vi "SysDef.Compile.vi"(8 "error in (no error)":errorcluster, 11 "Device Reference in":T1 format="%.0x") -> (0 "error out":errorcluster, 1 "Refs":T2(array[cluster]) {"VS Refs" format="%.0x"}, 2 "VS References":T3={"Name"="", "CAN"={"Interface"="", "Baud Rate"=0, "Diagnostic Protocol"=enum."GMLAN", "Transport Protocol"=enum."ISO TP - Normal Mode", "Transmit ID"=0, "Receive ID"=2, "Transmit Extension"=1, "Receive Extension"=255, "Receive UUDT ID"=0, "Enable Stream"=TRUE, "VW TP Channel ID"=1, "Fill Frame"=FALSE, "Fill Byte"=0, "Termination"=FALSE, "LIN Cluster"="", "NAD"=8, "IO Mode"=0, "Max DLC"=0, "FD Baud Rate"=2, "Timeout"=1, "FD ISO Mode"=0, "DoIP Address"="", "DoIP Source Address"=3584, "DoIP Dynamic Port"=TRUE, "DoIP Version"=2}, "986x"={"Enable"=FALSE, "RIO Device"="", "Bitfile"=path ""}, "Reads"=[], "Frames Lookup"=variant(enum16{"GMLAN", "KWP-2000", "UDS"} enum."GMLAN"), "Writes"=[], "DPIDs"=[], "DPID Lookup"=variant(u32 0), "DTC"={"Descriptor"={"DTC Byte Length"=1, "Status Byte Length"=1, "Add Data Byte Length"=1, "Byte Order"=enum."Motorola"}, "Value.Code"=[], "Value.String"=[], "Value.J2012String"=[], "Status.Code"=[], "Status.String"=[]}, "Created DTCs"=0, "Polls"=[], "Service Channels Status Lookup"=variant, "Trigger Lookup"=variant, "Security"={"Type"=enum."None", "Source DLL Path"=path "", "Target DLL Path"=path "", "Security Level"=1, "Static Master Key"="", "Max Key Length"=1, "Host IP Address"="", "ECU  Variant"=0, "Optional Parameter"=0}, "Initial Comm State"=FALSE} {"Writes"."Signals"."Byte Order" items=["Little Endian", "Big Endian"]; "Writes"."Signals"."Data Type" items=["Signed", "Unsigned", "IEEE Float"]; "CAN"."DoIP Version" items=["2010"=1, "2012"=2]; "CAN"."DoIP Source Address" format="%.0x"; "CAN"."FD ISO Mode" items=["ISO", "Non ISO", "ISO Legacy"]; "CAN"."IO Mode" items=["CAN 2.0", "CAN FD", "CAN FD+BRS"]; "CAN"."Fill Byte" format="%.0x"; "CAN"."VW TP Channel ID" format="%.0x"; "CAN"."Receive UUDT ID" format="%.0x"; "CAN"."Receive Extension" format="%.0x"; "CAN"."Transmit Extension" format="%.0x"; "CAN"."Receive ID" format="%.0x"; "CAN"."Transmit ID" format="%.0x"; "Reads"."Signals"."Byte Order" items=["Little Endian", "Big Endian"]; "Reads"."Signals"."Data Type" items=["Signed", "Unsigned", "IEEE Float"]}, 3 "Device Reference out":T1 format="%.0x")   [LabVIEW 2024, in "Diagnostics Addon System Explorer.lvlib"]
uses:
  Diagnostics Addon System Explorer.lvlib
  <vilib>/NI VeriStand/Custom Device API/Custom Device Item Ref.ctl
  Addon Shared/Types/SysDef.Compile.ctl
  Addon Shared/Types/CAN.ctl
  Addon Shared/Types/CAN.Interface.ctl
  Addon Shared/Types/Protocol.ctl
  Addon Shared/Types/Transport.ctl
  Addon Shared/Types/986x.ctl
  Addon Shared/Types/Frame.Compile.ctl
  Addon Shared/Types/Type.ctl
  Addon Shared/Types/Signal.ctl
  Addon Shared/Types/DPID.ctl
  Addon Shared/Types/DPID.Rate.ctl
  Addon Shared/Types/DTC.Settings.ctl
  Addon Shared/Types/DTC.Descriptor.ctl
  Addon Shared/Types/Poll.Compiled.ctl
  Addon Shared/Types/Security.ctl
  Addon Shared/Types/Security.Type.ctl
  Types/FG.Action.ctl
  ID.FG.vi
  Signals.Get.vi
  Type.FG.vi
  ServiceChannels.GetRefs.vi
  SettingChannels.GetRefs.vi
  Addon Shared/SubVIs/Frame.Get.Size.vi
  Addon Shared/SubVIs/LookupID.Create.vi
  DPID.FG.vi
  Security.FG.vi
  Signal.FG.vi
  Frame.GetSignalRefs.vi
  FileDependency.Create.vi
  Addon Shared/SubVIs/Constants.vi
  <vilib>/NI VeriStand/Custom Device Tools/Custom Device Utility Library/NI VeriStand - Search for Item by GUID.vi
  <vilib>/NI VeriStand/Custom Device Tools/Custom Device Utility Library/NI VeriStand - Search for Item by Name.vi
  <vilib>/NI VeriStand/Custom Device API/NI VeriStand - Get Item Children.vi
  <vilib>/NI/NI VeriStand Advanced SysDef API/SysDef API/SysDef.Property.Set.vi
  <vilib>/NI/NI VeriStand Advanced SysDef API/_SubVIs/SysDef.Property.Set.U32.vi
  <vilib>/NI VeriStand/Custom Device API/NI VeriStand - Get Item Property.vi
  <vilib>/NI VeriStand/Custom Device API/Get Item Property (U32).vi
  <vilib>/NI/NI VeriStand Advanced SysDef API/_SubVIs/SysDef.Property.Set.DBL.vi
  <vilib>/NI/NI VeriStand Advanced SysDef API/_SubVIs/SysDef.Property.Set.String.vi
  <vilib>/NI VeriStand/Custom Device API/Get Item Property (Double).vi
  <vilib>/NI VeriStand/Custom Device API/Get Item Property (String).vi
  <vilib>/NI VeriStand/Custom Device API/NI VeriStand - Get Custom Device Channel Data.vi
  <vilib>/NI VeriStand/Custom Device Tools/Custom Device Utility Library/NI VeriStand - Search for All Items by GUID.vi
  <vilib>/NI VeriStand/Custom Device API/Get Item Property (Variant).vi
  <vilib>/NI VeriStand/Custom Device API/Get Item Property (Boolean).vi
  <vilib>/NI VeriStand/Custom Device API/Get Item Property (U16).vi
  <vilib>/NI/NI VeriStand Advanced SysDef API/_SubVIs/SysDef.Property.Set.Variant.vi
  <vilib>/NI/NI VeriStand Advanced SysDef API/_SubVIs/SysDef.Property.Set.Boolean.vi
  <vilib>/NI/NI VeriStand Advanced SysDef API/_SubVIs/SysDef.Property.Set.U16.vi
  Service.EnumToGUID.vi
  <vilib>/NI VeriStand/Custom Device API/Get Item Property (Path).vi
  FileDependency.Get.Target Path.vi
  <vilib>/NI VeriStand/Custom Device API/Get Item Property (I32).vi
  <vilib>/NI/NI VeriStand Advanced SysDef API/SysDef API/SysDef.Property.Remove.vi
  <vilib>/NI/NI VeriStand Advanced SysDef API/_SubVIs/SysDef.Property.Set.Path.vi
  <vilib>/Utility/MD5Checksum.llb/MD5Checksum File.vi
  <vilib>/NI/NI VeriStand Advanced SysDef API/_SubVIs/SysDef.Property.Set.DependentFile.vi
  <vilib>/NI/NI VeriStand Advanced SysDef API/_SubVIs/SysDef.Property.Set.I32.vi
  <vilib>/NI/NI VeriStand Advanced SysDef API/_SubVIs/SysDef.Property.Set.U32.Array.vi
  <vilib>/NI VeriStand/Custom Device API/Get Item Property (U32 Array).vi
  Poll.FG.vi
  <vilib>/NI/NI VeriStand Advanced SysDef API/_SubVIs/SysDef.Property.Set.DBL.Array.vi
  <vilib>/NI/NI VeriStand Advanced SysDef API/_SubVIs/SysDef.Property.Set.String.Array.vi
  <vilib>/NI VeriStand/Custom Device API/Get Item Property (Double Array).vi
  <vilib>/NI VeriStand/Custom Device API/Get Item Property (String Array).vi
  <vilib>/NI VeriStand/Custom Device Tools/Custom Device Utility Library/Custom Device Utility Library.lvlib
  Addon Shared/Diagnostics Addon Shared.lvlib
  <vilib>/NI VeriStand/Custom Device API/Custom Device API.lvlib
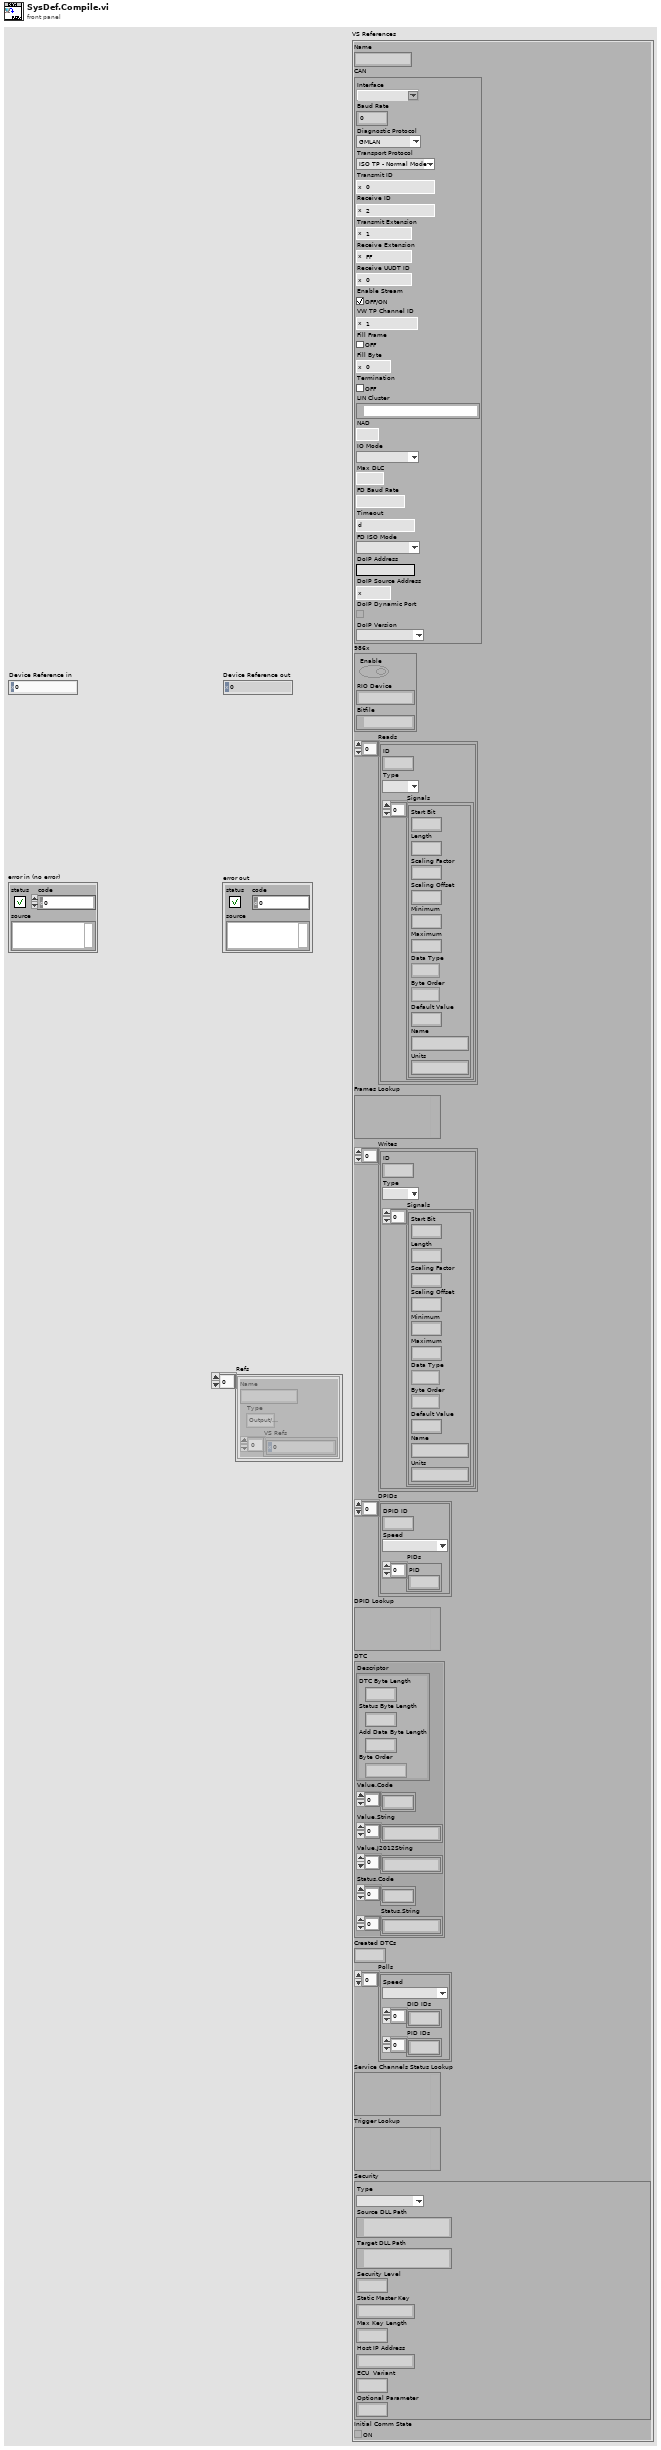
[diagram p1: front panel]
types:
  T1 = typedef "Custom Device API.lvlib/Custom Device Item Ref.ctl" = u64
  T2 = cluster{"Name":string, "Type":enum16{"Output/Write", "Input/Read", "Input/ReadWrite"}, "VS Refs":T1[]}[]
  T3 = typedef "Diagnostics Addon Shared.lvlib/SysDef.Compile.ctl" = cluster{"Name":string, "CAN":T4, "986x":T8, "Reads":T9[], "Frames Lookup":variant, "Writes":T9[], "DPIDs":T12[], "DPID Lookup":variant, "DTC":T14, "Created DTCs":u32, "Polls":T16[], "Service Channels Status Lookup":variant, "Trigger Lookup":variant, "Security":T17, "Initial Comm State":bool}
  T4 = typedef "Diagnostics Addon Shared.lvlib/CAN.ctl" = cluster{"Interface":T5, "Baud Rate":u64, "Diagnostic Protocol":T6, "Transport Protocol":T7, "Transmit ID":u32, "Receive ID":u32, "Transmit Extension":u8, "Receive Extension":u8, "Receive UUDT ID":u32, "Enable Stream":bool, "VW TP Channel ID":u32, "Fill Frame":bool, "Fill Byte":u8, "Termination":bool, "LIN Cluster":refnum<k21>, "NAD":u8, "IO Mode":u32, "Max DLC":u16, "FD Baud Rate":u64, "Timeout":u32, "FD ISO Mode":u32, "DoIP Address":string, "DoIP Source Address":u16, "DoIP Dynamic Port":bool, "DoIP Version":u16}
  T5 = typedef "Diagnostics Addon Shared.lvlib/CAN.Interface.ctl" = string
  T6 = typedef "Diagnostics Addon Shared.lvlib/Protocol.ctl" = enum16{"GMLAN", "KWP-2000", "UDS", "User-Defined"}
  T7 = typedef "Diagnostics Addon Shared.lvlib/Transport.ctl" = enum16{"ISO TP - Normal Mode", "ISO TP - Mixed Mode", "VW TP 2.0", "Diagnostics on IP", "ISO TP LIN"}
  T8 = typedef "Diagnostics Addon Shared.lvlib/986x.ctl" = cluster{"Enable":bool, "RIO Device":string, "Bitfile":path}
  T9 = typedef "Diagnostics Addon Shared.lvlib/Frame.Compile.ctl" = cluster{"ID":u32, "Type":T10, "Signals":T11[]}
  T10 = typedef "Diagnostics Addon Shared.lvlib/Type.ctl" = enum16{"DID", "CDID", "PID", "CPID", "Read Memory", "Write Memory", "IO Control", "Routine Start", "Routine Request", "Routine Stop", "User Defined", "DTC Control", "Clear DTCs", "Read DTCs", "Start DTCs", "DTC Change Count", "Tester Present", "Unlock ECU", "Reset ECU", "Diag Session Control", "Communication Control", "DPID Control", "Poll Control", "Diag Comm Port Control"}
  T11 = typedef "Diagnostics Addon Shared.lvlib/Signal.ctl" = cluster{"Start Bit":u32, "Length":u32, "Scaling Factor":dbl, "Scaling Offset":dbl, "Minimum":dbl, "Maximum":dbl, "Data Type":u32, "Byte Order":u32, "Default Value":dbl, "Name":string, "Units":string}
  T12 = typedef "Diagnostics Addon Shared.lvlib/DPID.ctl" = cluster{"DPID ID":u8, "Speed":T13, "PIDs":u16[]}
  T13 = typedef "Diagnostics Addon Shared.lvlib/DPID.Rate.ctl" = enum16{"Slow", "Medium", "Fast"}
  T14 = typedef "Diagnostics Addon Shared.lvlib/DTC.Settings.ctl" = cluster{"Descriptor":T15, "Value.Code":dbl[], "Value.String":string[], "Value.J2012String":string[], "Status.Code":dbl[], "Status.String":string[]}
  T15 = typedef "Diagnostics Addon Shared.lvlib/DTC.Descriptor.ctl" = cluster{"DTC Byte Length":i32, "Status Byte Length":i32, "Add Data Byte Length":i32, "Byte Order":enum16{"Motorola", "Intel"}}
  T16 = typedef "Diagnostics Addon Shared.lvlib/Poll.Compiled.ctl" = cluster{"Speed":T13, "DID IDs":u32[], "PID IDs":u32[]}
  T17 = typedef "Diagnostics Addon Shared.lvlib/Security.ctl" = cluster{"Type":T18, "Source DLL Path":path, "Target DLL Path":path, "Security Level":u32, "Static Master Key":string, "Max Key Length":u32, "Host IP Address":string, "ECU  Variant":i8, "Optional Parameter":i8}
  T18 = typedef "Diagnostics Addon Shared.lvlib/Security.Type.ctl" = enum16{"None", "SeedKey DLL", "MasterKey (Channel)", "MasterKey (Static)", "SeedKey DLL (Windows)"}
  T19 = enum16{"Output/Write", "Input/Read", "Input/ReadWrite"}
  T20 = cluster{"Name":string, "Type":enum16{"Output/Write", "Input/Read", "Input/ReadWrite"}, "VS Refs":T1[]}
  T21 = typedef "Diagnostics Addon System Explorer.lvlib/FG.Action.ctl" = enum16{"Get", "Set"}
  T22 = typedef "Diagnostics Addon System Explorer.lvlib/Service.Export.ctl" = cluster{"Signal.Cmd.Refs":T23[], "Signal.Cmd.Info":T9[], "Signal.Resp.Refs":T23[], "Signal.Resp.Info":T9[], "Trigger.Refs":T23[], "Status.Refs":T23[], "Settings.Refs":T23[]}
  T23 = typedef "Diagnostics Addon System Explorer.lvlib/Frame.Ref.ctl" = cluster{"Type":T10, "ID":u32, "Signal Refs":T1[]}
  T24 = typedef "Custom Device API.lvlib/Custom Device Item Info.ctl" = cluster{"Name":string, "Is Channel":bool, "GUID":string, "Is Waveform":bool}
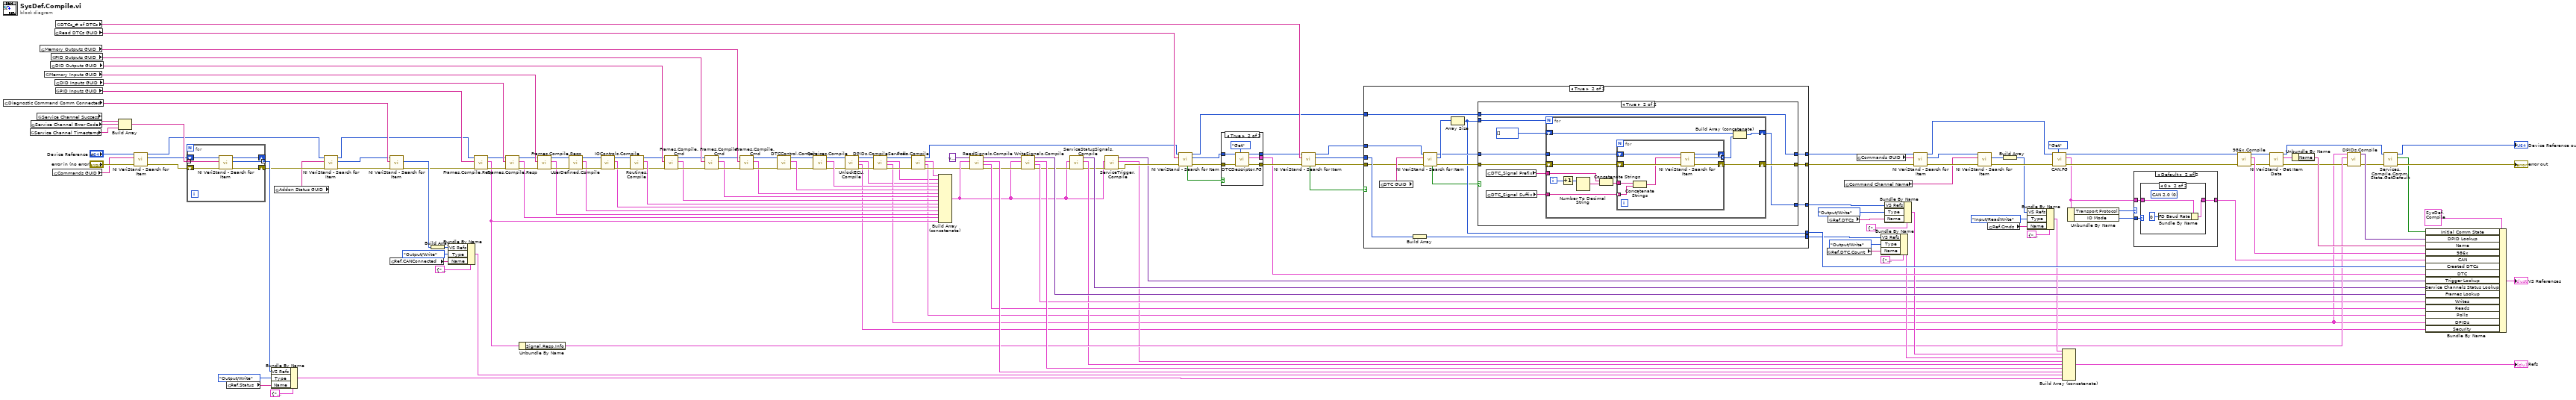
[diagram p0: block diagram]
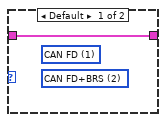
[diagram p3: hidden frame]
diagram:
  n1 = global read "Constants.vi" "Diagnostic Command Comm Connected"() -> (w76:string)
  n2 = global read "Constants.vi" "Service Channel Timestamp"() -> (w19:string)
  n3 = global read "Constants.vi" "Service Channel Error Code"() -> (w20:string)
  n4 = global read "Constants.vi" "Service Channel Success"() -> (w18:string)
  n5 = global read "Constants.vi" "Memory Outputs GUID"() -> (w133:string)
  n6 = global read "Constants.vi" "Memory Inputs GUID"() -> (w132:string)
  n7 = global read "Constants.vi" "DID Outputs GUID"() -> (w114:string)
  n8 = global read "Constants.vi" "PID Outputs GUID"() -> (w152:string)
  n9 = global read "Constants.vi" "Commands GUID"() -> (w67:string)
  n10 = global read "Constants.vi" "Read DTCs GUID"() -> (w156:string)
  n11 = global read "Constants.vi" "DID Inputs GUID"() -> (w153:string)
  n12 = global read "Constants.vi" "PID Inputs GUID"() -> (w151:string)
  n13 = global read "Constants.vi" "DTCs_# of DTCs"() -> (w155:string)
  n14 = Build Array(w18, w20, w19) -> (w118:string[])
  n15 = call-poly <vilib>:"NI VeriStand - Search for Item.vi"("error in"="error in (no error)", "Item GUID"=w67, "Section Ref in"="Device Reference in") -> ("error out"=w11:errorcluster, "Item Ref"=w10:T1, "Section Ref out"=w15:T1)  [unwired: 5 in, 1 out]
  n16 = for {
    tunnel: w118 -> [w160] mode=indexing
    tunnel: [w159] -> w96 mode=indexing
    shift-right: [w158] -> w17
    shift-left: w11 -> [w162]
    shift-right: [w157] -> _
    shift-left: w10 -> [w161]
    n17 = call-poly <vilib>:"NI VeriStand - Search for Item.vi"("error in"=w162, "Item Name"=w160, "Section Ref in"=w161) -> ("error out"=w158:errorcluster, "Item Ref"=w159:T1, "Section Ref out"=w157:T1)  [unwired: 5 in, 1 out]
  }
  n18 = global read "Constants.vi" "Ref.Status"() -> (w104:string)
  n19 = Bundle By Name(cluster=T20 {"Name"="", "Type"=enum."Output/Write", "VS Refs"=[]} ("Group"), "VS Refs"=w96, "Type"=T19."Output/Write", "Name"=w104) -> (w92:T20)
  n20 = global read "Constants.vi" "Addon Status GUID"() -> (w12:string)
  n21 = call-poly <vilib>:"NI VeriStand - Search for Item.vi"("error in"=w17, "Item GUID"=w12, "Section Ref in"=w15) -> ("error out"=w16:errorcluster, "Item Ref"=w13:T1, "Section Ref out"=w14:T1)  [unwired: 5 in, 1 out]
  n22 = call-poly <vilib>:"NI VeriStand - Search for Item.vi"("error in"=w16, "Item Name"=w76, "Section Ref in"=w13) -> ("error out"=w71:errorcluster, "Item Ref"=w73:T1)  [unwired: 5 in, 2 out]
  n23 = global read "Constants.vi" "Ref.CANConnected"() -> (w75:string)
  n24 = Build Array(w73) -> (w72:T1[])
  n25 = Bundle By Name(cluster=T20 {"Name"="", "Type"=enum."Output/Write", "VS Refs"=[]} ("Group"), "VS Refs"=w72, "Type"=T19."Output/Write", "Name"=w75) -> (w66:T20)
  n26 = call "Frames.Compile.Resp.vi"("error in (no error)"=w71, "GUID"=w151, "Section Ref in"=w14) -> ("error out"=w126:errorcluster, "Settings"=w61:T22, "Section Ref out"=w131:T1)  [unwired: 6 in]
  n27 = call "Frames.Compile.Resp.vi"("error in (no error)"=w126, "GUID"=w153, "Section Ref in"=w131) -> ("error out"=w127:errorcluster, "Settings"=w62:T22, "Section Ref out"=w130:T1)  [unwired: 6 in]
  n28 = Unbundle By Name(w61) -> ("Signal.Resp.Info"=w65:T9[])
  n29 = call "Frames.Compile.Resp.vi"("error in (no error)"=w127, "GUID"=w132, "Section Ref in"=w130) -> ("error out"=w112:errorcluster, "Settings"=w63:T22, "Section Ref out"=w113:T1)  [unwired: 6 in]
  n30 = call "UserDefined.Compile.vi"("error in (no error)"=w112, "Section Ref in"=w113) -> ("error out"=w111:errorcluster, "Settings"=w59:T22, "Section Ref out"=w110:T1)  [unwired: 7 in]
  n31 = call "IOControls.Compile.vi"("error in (no error)"=w111, "Section Ref in"=w110) -> ("error out"=w128:errorcluster, "Settings"=w58:T22, "Section Ref out"=w129:T1)  [unwired: 7 in]
  n32 = call "Routines.Compile.vi"("error in (no error)"=w128, "Section Ref in"=w129) -> ("error out"=w52:errorcluster, "Settings"=w57:T22, "Section Ref out"=w51:T1)  [unwired: 7 in]
  n33 = call "Frames.Compile.Cmd.vi"("error in (no error)"=w52, "GUID"=w114, "Section Ref in"=w51) -> ("error out"=w115:errorcluster, "Settings"=w53:T22, "Section Ref out"=w116:T1)  [unwired: 6 in]
  n34 = call "Frames.Compile.Cmd.vi"("error in (no error)"=w115, "GUID"=w152, "Section Ref in"=w116) -> ("error out"=w120:errorcluster, "Settings"=w54:T22, "Section Ref out"=w123:T1)  [unwired: 6 in]
  n35 = call "Frames.Compile.Cmd.vi"("error in (no error)"=w120, "GUID"=w133, "Section Ref in"=w123) -> ("error out"=w121:errorcluster, "Settings"=w55:T22, "Section Ref out"=w122:T1)  [unwired: 6 in]
  n36 = call "DTCControl.Compile.vi"("error in (no error)"=w121, "Section Ref in"=w122) -> ("error out"=w41:errorcluster, "Settings"=w56:T22, "Section Ref out"=w40:T1)  [unwired: 7 in]
  n37 = call "Services.Compile.vi"("error in (no error)"=w41, "Section Ref in"=w40) -> ("error out"=w25:errorcluster, "Settings"=w39:T22[], "Section Ref out"=w26:T1)  [unwired: 7 in]
  n38 = call "UnlockECU.Compile.vi"("error in (no error)"=w25, "Section Ref in"=w26) -> ("error out"=w24:errorcluster, "Security"=w21:T17, "Settings"=w22:T22[], "Section Ref out"=w23:T1)  [unwired: 6 in]
  n39 = call "DPIDs.CompileServices.vi"("error in (no error)"=w24, "Section Ref in"=w23) -> ("error out"=w32:errorcluster, "DPIDs Settings"=w28:T12[], "Settings"=w30:T22, "Section Ref out"=w31:T1)  [unwired: 6 in]
  n40 = call "Polls.Compile.vi"("error in (no error)"=w32, "Section Ref in"=w31) -> ("error out"=w36:errorcluster, "Poll Settings"=w33:T16[], "Service Channels"=w34:T22[], "Section Ref out"=w35:T1)  [unwired: 6 in]
  n41 = Build Array (concatenate)(w34, w30, w22, w39, w56, w55, w54, w53, w57, w58, w59, w63, w62, w61) -> (w44:T22[])
  n42 = call "ReadSignals.Compile.vi"("error in (no error)"=w36, "Settings"=w44, "Lookups in"=variant) -> ("error out"=w50:errorcluster, "Signal Info"=w64:T9[], "Refs"=w93:T20, "Lookups"=w101:variant)  [unwired: 5 in]
  n43 = call "WriteSignals.Compile.vi"("error in (no error)"=w50, "Settings"=w44, "Lookup In"=w101) -> ("error out"=w49:errorcluster, "Signal Info"=w60:T9[], "Refs"=w94:T20, "Lookup"=w100:variant)  [unwired: 5 in]
  n44 = call "ServiceStatusSignals.Compile.vi"("error in (no error)"=w49, "Settings"=w44) -> ("error out"=w46:errorcluster, "Refs"=w48:T20, "Status Lookup"=w47:variant)  [unwired: 7 in]
  n45 = call "ServiceTrigger.Compile.vi"("error in (no error)"=w46, "Settings"=w44) -> ("error out"=w45:errorcluster, "Refs"=w43:T2, "Trigger Lookup"=w42:variant)  [unwired: 7 in]
  n46 = call-poly <vilib>:"NI VeriStand - Search for Item.vi"("error in"=w45, "Item GUID"=w156, "Section Ref in"=w35) -> ("error out"=w147:errorcluster, "Item Ref"=w145:T1, "Section Ref out"=w117:T1, "Found"=w107:bool)  [unwired: 5 in]
  n47 = case shown="True" w107 {
    tunnel: w147 -> [w164 w169]
    tunnel: [w164 w168] -> w146
    tunnel: w145 -> [w163 w167]
    tunnel: [w163 w166] -> w144
    tunnel: [_ w165] -> w143
    frame False {
    }
    frame True {
      n48 = call "DTCDescriptor.FG.vi"("Action"=FG.Action."Get", "error in (no error)"=w169, "Device Item Ref in"=w167) -> ("error out"=w168:errorcluster, "DTC descriptor"=w165:T14, "Device Item Ref out"=w166:T1)  [unwired: 6 in]
    }
  }
  n49 = call-poly <vilib>:"NI VeriStand - Search for Item.vi"("error in"=w146, "Item Name"=w155, "Section Ref in"=w144) -> ("error out"=w149:errorcluster, "Item Ref"=w150:T1, "Section Ref out"=w109:T1, "Found"=w106:bool)  [unwired: 5 in]
  n50 = case shown="True" w106 {
    tunnel: w150 -> [_ w176]
    tunnel: w149 -> [w171 w175]
    tunnel: [_ w186] -> w86
    tunnel: [w171 w185] -> w125
    tunnel: [w172 w184] -> w124
    tunnel: w117 -> [w172 w174]
    tunnel: w109 -> [_ w181]
    tunnel: [_ w178] -> w108
    tunnel: [_ w173] -> w82
    frame False {
    }
    frame True {
      n51 = global read "Constants.vi" "DTC GUID"() -> (w179:string)
      n52 = Build Array(w176) -> (w173:T1[])
      n53 = call-poly <vilib>:"NI VeriStand - Search for Item.vi"("error in"=w175, "Item GUID"=w179, "Section Ref in"=w181) -> ("error out"=w183:errorcluster, "Item Refs"=w182:T1[], "Section Ref out"=w180:T1, "Found"=w177:bool)  [unwired: 5 in]
      n54 = Array Size(array=w182) -> (size(s)=w178:i32)
      n55 = case shown="True" w177 {
        tunnel: [_ w189] -> w186
        tunnel: [w187 w191] -> w185
        tunnel: [w188 w190] -> w184
        tunnel: w174 -> [w188 w190]
        tunnel: w183 -> [w187 w194]
        tunnel: w180 -> [_ w193]
        tunnel: w178 -> [_ w192]
        frame False {
        }
        frame True {
          n56 = global read "Constants.vi" "DTC_Signal Prefix"() -> (w197:string)
          n57 = global read "Constants.vi" "DTC_Signal Suffix"() -> (w196:string[])
          n58 = for {
            N: w192 -> [_]
            tunnel: w193 -> [w209]
            shift-right: [w207] -> w191
            shift-left: w194 -> [w208]
            tunnel: w196 -> [w202]
            tunnel: w197 -> [w201]
            shift-right: [w198] -> w189
            shift-left: T1[] [] -> [w200]
            i -> [w204]
            n59 = Increment(x=w204) -> (x+1=w206:i32)
            n60 = Number To Decimal String(number=w206) -> (decimal integer string=w205:string)  [unwired: 1 in]
            n61 = Concatenate Strings(w201, w205) -> (w203:string)
            n62 = for {
              shift-right: [w216] -> _
              shift-left: w209 -> [w217]
              shift-right: [w214] -> w207
              shift-left: w208 -> [w215]
              tunnel: w202 -> [w213] mode=indexing
              tunnel: w203 -> [w212]
              tunnel: [w210] -> w199 mode=indexing
              n63 = Concatenate Strings(w212, w213) -> (w211:string)
              n64 = call-poly <vilib>:"NI VeriStand - Search for Item.vi"("error in"=w215, "Item Name"=w211, "Section Ref in"=w217) -> ("error out"=w214:errorcluster, "Item Ref"=w210:T1, "Section Ref out"=w216:T1)  [unwired: 5 in, 1 out]
            }
            n65 = Build Array (concatenate)(w200, w199) -> (w198:T1[])
          }
        }
      }
    }
  }
  n66 = global read "Constants.vi" "Ref.DTC.Count"() -> (w84:string)
  n67 = global read "Constants.vi" "Ref.DTCs"() -> (w89:string)
  n68 = global read "Constants.vi" "Command Channel Name"() -> (w78:string)
  n69 = global read "Constants.vi" "Commands GUID"() -> (w154:string)
  n70 = Bundle By Name(cluster=T20 {"Name"="", "Type"=enum."Output/Write", "VS Refs"=[]} ("Group"), "VS Refs"=w82, "Type"=T19."Output/Write", "Name"=w84) -> (w81:T20)
  n71 = Bundle By Name(cluster=T20 {"Name"="", "Type"=enum."Output/Write", "VS Refs"=[]} ("Group"), "VS Refs"=w86, "Type"=T19."Output/Write", "Name"=w89) -> (w87:T20)
  n72 = call-poly <vilib>:"NI VeriStand - Search for Item.vi"("error in"=w125, "Item GUID"=w154, "Section Ref in"=w124) -> ("error out"=w80:errorcluster, "Item Ref"=w79:T1, "Section Ref out"=w37:T1)  [unwired: 5 in, 1 out]
  n73 = call-poly <vilib>:"NI VeriStand - Search for Item.vi"("error in"=w80, "Item Name"=w78, "Section Ref in"=w79) -> ("error out"=w38:errorcluster, "Item Ref"=w77:T1)  [unwired: 5 in, 2 out]
  n74 = global read "Constants.vi" "Ref.Cmds"() -> (w98:string)
  n75 = Build Array(w77) -> (w27:T1[])
  n76 = Bundle By Name(cluster=T20 {"Name"="", "Type"=enum."Output/Write", "VS Refs"=[]} ("Group"), "VS Refs"=w27, "Type"=T19."Input/ReadWrite", "Name"=w98) -> (w95:T20)
  n77 = call "CAN.FG.vi"("Action"=FG.Action."Get", "error in (no error)"=w38, "Device Item Ref in"=w37) -> ("error out"=w142:errorcluster, "Diagnostics Basic Configuration"=w8:T4, "Device Item Ref out"=w141:T1)  [unwired: 6 in]
  n78 = Build Array (concatenate)(w95, w87, w81, w43, w48, w94, w93, w66, w92) -> (→"Refs":T2)
  n79 = Unbundle By Name(w8) -> ("Transport Protocol"=w6:T7, "IO Mode"=w9:u32)
  n80 = case shown="Default" w6 {
    tunnel: w9 -> [_ w221]
    tunnel: w8 -> [w218 w220]
    tunnel: [w218 w219] -> w7
    frame "VW TP 2.0".."ISO TP LIN" {
    }
    frame Default {
      n81 = case shown="0" w221 {
        tunnel: w220 -> [w222 w225]
        tunnel: [w222 w224] -> w219
        frame Default {
          (unwired) u32 2 items=["CAN 2.0", "CAN FD", "CAN FD+BRS"] ("IO Mode")
          (unwired) u32 1 items=["CAN 2.0", "CAN FD", "CAN FD+BRS"] ("IO Mode")
        }
        frame 0 {
          (unwired) u32 0 items=["CAN 2.0", "CAN FD", "CAN FD+BRS"] ("IO Mode")
          n82 = Bundle By Name(cluster=w225, "FD Baud Rate"=u64 0) -> (w224:T4)
        }
      }
    }
  }
  n83 = call "986x.Compile.vi"("error in (no error)"=w142, "Item Ref in"=w141) -> ("error out"=w137:errorcluster, "986x Support"=w140:T8, "Item Ref out"=w136:T1)  [unwired: 7 in]
  n84 = call <vilib>:"NI VeriStand - Get Item Data.vi"("error in (no error)"=w137, "Item Ref in"=w136) -> ("error out"=w29:errorcluster, "Item Info"=w138:T24, "Item Ref out"=w3:T1)  [unwired: 6 in, 1 out]
  n85 = Unbundle By Name(w138) -> ("Name"=w135:string)
  n86 = call "DPIDs.Compile.vi"("error in (no error)"=w29, "PIDs"=w65, "DPIDs"=w28) -> ("error out"=w5:errorcluster, "Lookup Table"=w134:variant)  [unwired: 7 in]
  n87 = call "Services.Compile.Comm.State.GetDefault.vi"("error in (no error)"=w5, "Section Ref in"=w3) -> ("error out"=→"error out":errorcluster, "Initial Comm State"=w1:bool, "Section Ref out"=→"Device Reference out":T1)  [unwired: 7 in]
  n88 = Bundle By Name(cluster=T3 {"Name"="", "CAN"={"Interface"="", "Baud Rate"=0, "Diagnostic Protocol"=enum."GMLAN", "Transport Protocol"=enum."ISO TP - Normal Mode", "Transmit ID"=0, "Receive ID"=2, "Transmit Extension"=1, "Receive Extension"=255, "Receive UUDT ID"=0, "Enable Stream"=TRUE, "VW TP Channel ID"=1, "Fill Frame"=FALSE, "Fill Byte"=0, "Termination"=FALSE, "LIN Cluster"="", "NAD"=8, "IO Mode"=0, "Max DLC"=0, "FD Baud Rate"=2, "Timeout"=1, "FD ISO Mode"=0, "DoIP Address"="", "DoIP Source Address"=3584, "DoIP Dynamic Port"=TRUE, "DoIP Version"=2}, "986x"={"Enable"=FALSE, "RIO Device"="", "Bitfile"=path ""}, "Reads"=[], "Frames Lookup"=variant(enum16{"GMLAN", "KWP-2000", "UDS"} enum."GMLAN"), "Writes"=[], "DPIDs"=[], "DPID Lookup"=variant(u32 0), "DTC"={"Descriptor"={"DTC Byte Length"=1, "Status Byte Length"=1, "Add Data Byte Length"=1, "Byte Order"=enum."Motorola"}, "Value.Code"=[], "Value.String"=[], "Value.J2012String"=[], "Status.Code"=[], "Status.String"=[]}, "Created DTCs"=0, "Polls"=[], "Service Channels Status Lookup"=variant, "Trigger Lookup"=variant, "Security"={"Type"=enum."None", "Source DLL Path"=path "", "Target DLL Path"=path "", "Security Level"=1, "Static Master Key"="", "Max Key Length"=1, "Host IP Address"="", "ECU  Variant"=0, "Optional Parameter"=0}, "Initial Comm State"=FALSE} ("VS References"), "Initial Comm State"=w1, "DPID Lookup"=w134, "Name"=w135, "986x"=w140, "CAN"=w7, "Created DTCs"=w108, "DTC"=w143, "Trigger Lookup"=w42, "Service Channels Status Lookup"=w47, "Frames Lookup"=w100, "Writes"=w60, "Reads"=w64, "Polls"=w33, "DPIDs"=w28, "Security"=w21) -> (→"VS References":T3)
